vi "Test String Subset.vi"(8 "error in (no error)":errorcluster) -> (0 "error out":errorcluster, 3 "Pass?":bool)   [LabVIEW 2020]
uses:
  G-Unicode/Types/UTF-8 String/UTF-8 String.lvclass/UTF-8 String.ctl
  6c3bdbaa-dd8a-4d7a-a6b3-47bb84b7ab58.vi
  264a07c0-f4c2-4ea3-88ef-a13d84b4d497.vi
  45aec575-2979-4ee1-8716-e0589e8f3a80.vi
  310073a2-a64f-4bb1-b41b-518da9507cbb.vi
  52367a98-e987-492e-8e34-06f004b52f76.vi
  0032c660-e719-47bc-bfae-3eb3c0e15da0.vi
  908b0875-7fce-4a01-b2dd-ed181c2719e3.vi
  e45cf646-96a9-420e-b517-089b6751d525.vi
  G-Unicode/Private/Conversion/String as Encoded String.vi
  G-Unicode/Private/Conversion/Polymorphic VIs/String as Encoded String (UTF-8 String).vi
  G-Unicode/Private/Library/gu_string_subset.vi
  264a07c0-f4c2-4ea3-88ef-a13d84b4d497.vi/3a31b270-3bb6-4c58-a256-c5fcc2c98f09.vi
  264a07c0-f4c2-4ea3-88ef-a13d84b4d497.vi/0ec5df2d-ef9b-4f84-a6a8-ffcedd45c4dc.vi
  310073a2-a64f-4bb1-b41b-518da9507cbb.vi/3a31b270-3bb6-4c58-a256-c5fcc2c98f09.vi
  310073a2-a64f-4bb1-b41b-518da9507cbb.vi/0ec5df2d-ef9b-4f84-a6a8-ffcedd45c4dc.vi
  G-Unicode/Private/Conversion/Polymorphic VIs/String as Encoded String (LabVIEW String).vi
  0032c660-e719-47bc-bfae-3eb3c0e15da0.vi/3a31b270-3bb6-4c58-a256-c5fcc2c98f09.vi
  0032c660-e719-47bc-bfae-3eb3c0e15da0.vi/0ec5df2d-ef9b-4f84-a6a8-ffcedd45c4dc.vi
  e45cf646-96a9-420e-b517-089b6751d525.vi/3a31b270-3bb6-4c58-a256-c5fcc2c98f09.vi
  e45cf646-96a9-420e-b517-089b6751d525.vi/0ec5df2d-ef9b-4f84-a6a8-ffcedd45c4dc.vi
  G-Unicode/Types/UTF-8 String/Read Encoded UTF-8 String.vi
  G-Unicode/Private/Memory/Copy String.vi
  G-Unicode/Private/Library/Result To Error.vi
  G-Unicode/Private/Conversion/Text as Encoded String.vi
  G-Unicode/Private/Conversion/Polymorphic VIs/Text as Encoded String (UTF-8 String).vi
  G-Unicode/Private/Conversion/Text to UTF-8.vi
  G-Unicode/Private/Conversion/Polymorphic VIs/Text to UTF-8 (LabVIEW String).vi
  G-Unicode/Private/Conversion/Polymorphic VIs/Text as Encoded String (LabVIEW String).vi
  G-Unicode/Private/Memory/Copy String.vi/4d47babd-4a2d-4eb7-b91b-7e707d692665.vi
  G-Unicode/Private/Library/gu_free.vi
  <vilib>/Utility/error.llb/Error Cluster From Error Code.vi
  G-Unicode/Types/UTF-8 String/UTF-8 String.lvclass
  8f41635d-b67f-4b6a-9ef1-d352021ab77f.vi
  G-Unicode/Unicode/Controls/String Encoding.ctl
  G-Unicode/G-Unicode.lvlib
  3ab6bfcf-5bba-49b8-9409-711e23355faa.vi
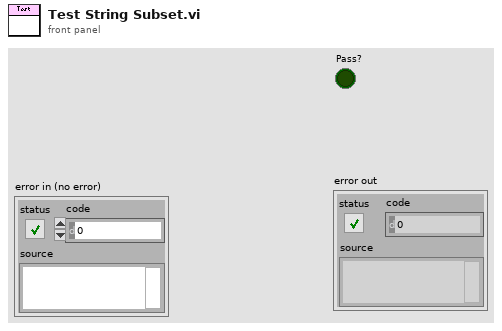
[diagram p1: front panel]
types:
  T1 = typedef "G-Unicode.lvlib/String Encoding.ctl" = enum16{"ANSI", "UTF-8", "UTF-16LE", "UTF-16BE", "Unknown"}
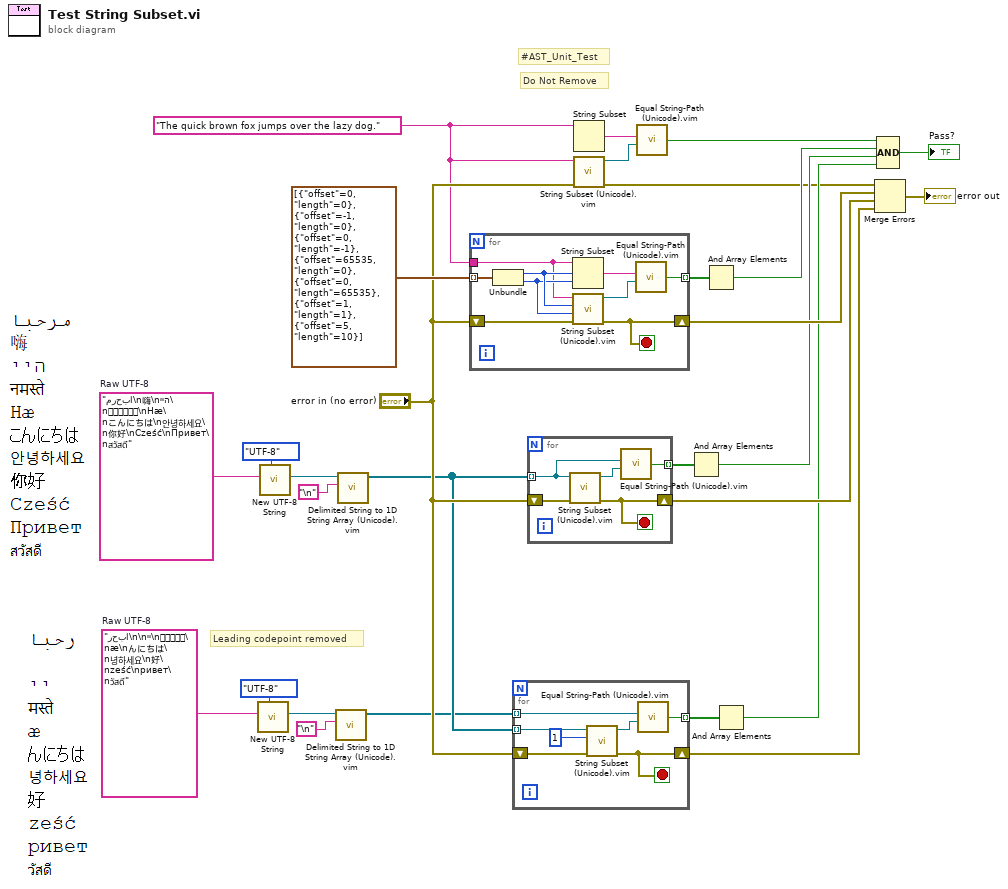
[diagram p0: block diagram]
diagram:
  w2 = "رحبا\n\nיי\nमस्ते\næ\nんにちは\n녕하세요\n好\nześć\nривет\nวัสดี"  # Raw UTF-8
  w11 = "The quick brown fox jumps over the lazy dog." ("string")
  w7 = "مرحبا\n嗨\nהיי\nनमस्ते\nHæ\nこんにちは\n안녕하세요\n你好\nCześć\nПривет\nสวัสดี"  # Raw UTF-8
  # "Leading codepoint removed"
  # "Do Not Remove"
  # "#AST_Unit_Test"
  n1 = call "New UTF-8 String.vi"("Input Encoding (ANSI)"=String_Encoding."UTF-8", "String"=w2) -> ("UTF-8 String"=w4:refnum<class "UTF-8 String.lvclass">)  [unwired: 8 in, 1 out]
  n2 = call "New UTF-8 String.vi"("Input Encoding (ANSI)"=String_Encoding."UTF-8", "String"=w7) -> ("UTF-8 String"=w9:refnum<class "UTF-8 String.lvclass">)  [unwired: 8 in, 1 out]
  n3 = call "Delimited String to 1D String Array (Unicode).vim"("Delimiter (tab)"="\n", "Delimited String"=w4) -> ("String Array"=w1:refnum<class "UTF-8 String.lvclass">[])  [unwired: 8 in, 1 out]
  n4 = call "Delimited String to 1D String Array (Unicode).vim"("Delimiter (tab)"="\n", "Delimited String"=w9) -> ("String Array"=w6:refnum<class "UTF-8 String.lvclass">[])  [unwired: 8 in, 1 out]
  n5 = for {
    tunnel: [w35] -> w22 mode=indexing
    shift-right: [w36] -> w28
    shift-left: "error in (no error)" -> [w37]
    tunnel: w11 -> [w29]
    tunnel: cluster{"offset":i32, "length":i32}[] [{"offset"=0, "length"=0}, {"offset"=-1, "length"=0}, {"offset"=0, "length"=-1}, {"offset"=65535, "length"=0}, {"offset"=0, "length"=65535}, {"offset"=1, "length"=1}, {"offset"=5, "length"=10}] -> [w33] mode=indexing
    stop <- w36 stop-if-true
    n6 = Unbundle(w33) -> ("offset"=w32:i32, "length"=w31:i32)
    n7 = String Subset(string=w29, offset (0)=w32, length (rest)=w31) -> (substring=w30:string)
    n8 = call "String Subset (Unicode).vim"("error in"=w37, "Length (rest)"=w31, "Offset (0)"=w32, "String"=w29) -> ("error out"=w36:errorcluster, "Substring"=w34:refnum<class "UTF-8 String.lvclass">)  [unwired: 6 in]
    n9 = call "Equal String-Path (Unicode).vim"("y"=w34, "x"=w30) -> ("Equal?"=w35:bool)  [unwired: 7 in, 1 out]
  }
  n10 = for {
    tunnel: w6 -> [w43] mode=indexing
    tunnel: [w42] -> w16 mode=indexing
    shift-right: [w41] -> w14
    shift-left: "error in (no error)" -> [w40]
    tunnel: w1 -> [w38] mode=indexing
    stop <- w41 stop-if-true
    n11 = call "String Subset (Unicode).vim"("error in"=w40, "Offset (0)"=1, "String"=w43) -> ("error out"=w41:errorcluster, "Substring"=w44:refnum<class "UTF-8 String.lvclass">)  [unwired: 7 in]
    n12 = call "Equal String-Path (Unicode).vim"("y"=w44, "x"=w38) -> ("Equal?"=w42:bool)  [unwired: 7 in, 1 out]
  }
  n13 = for {
    tunnel: w6 -> [w45] mode=indexing
    tunnel: [w48] -> w20 mode=indexing
    shift-right: [w47] -> w18
    shift-left: "error in (no error)" -> [w46]
    stop <- w47 stop-if-true
    n14 = call "String Subset (Unicode).vim"("error in"=w46, "String"=w45) -> ("error out"=w47:errorcluster, "Substring"=w49:refnum<class "UTF-8 String.lvclass">)  [unwired: 8 in]
    n15 = call "Equal String-Path (Unicode).vim"("y"=w49, "x"=w45) -> ("Equal?"=w48:bool)  [unwired: 7 in, 1 out]
  }
  n16 = String Subset(string=w11) -> (substring=w13:string)  [unwired: 2 in]
  n17 = call "String Subset (Unicode).vim"("error in"="error in (no error)", "String"=w11) -> ("error out"=w12:errorcluster, "Substring"=w26:refnum<class "UTF-8 String.lvclass">)  [unwired: 8 in]
  n18 = call "Equal String-Path (Unicode).vim"("y"=w26, "x"=w13) -> ("Equal?"=w25:bool)  [unwired: 7 in, 1 out]
  n19 = And Array Elements(Boolean array=w20) -> (logical AND=w19:bool)
  n20 = And Array Elements(Boolean array=w22) -> (logical AND=w21:bool)
  n21 = And Array Elements(Boolean array=w16) -> (logical AND=w15:bool)
  n22 = Merge Errors(w12, w28, w18, w14) -> (→"error out":errorcluster)
  n23 = Compound Arithmetic op=AND(w25, w21, w19, w15) -> (→"Pass?":bool)
